vi "UDP Refresh Packet Sizes.vi"(8 "error in (no error)":errorcluster, 10 "UDP UI References in":T2, 11 "node References":T1) -> (0 "error out":errorcluster, 2 "UDP UI References out":T2, 3 "node References out":T1)   [LabVIEW 2015, in "E2E Tag Exchange editor node.lvclass"]
uses:
  E2E Tag Exchange editor node.lvclass
  UDP UI References.ctl
  object references.ctl
  <vilib>/NI/DCAF/Tag Editor Core/Configuration Editor/Classes/Engine Parent/Engine Parent Editor Node.lvclass
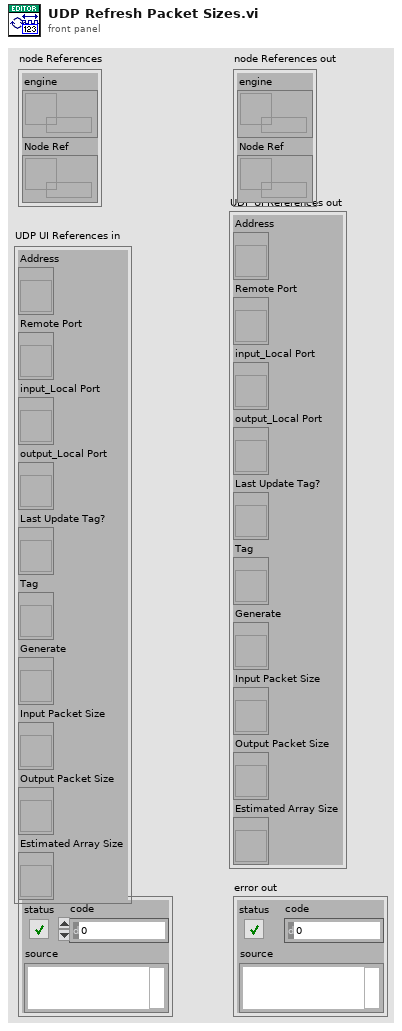
[diagram p1: front panel]
types:
  T1 = typedef "E2E Tag Exchange editor node.lvclass/object references.ctl" = cluster{"engine":refnum<data-value>, "Node Ref":refnum<data-value>}
  T2 = typedef "E2E Tag Exchange editor node.lvclass/UDP UI References.ctl" = cluster{"Address":refnum<vi>, "Remote Port":refnum<vi>, "input_Local Port":refnum<vi>, "output_Local Port":refnum<vi>, "Last Update Tag?":refnum<vi>, "Tag":refnum<vi>, "Generate":refnum<vi>, "Input Packet Size":refnum<vi>, "Output Packet Size":refnum<vi>, "Estimated Array Size":refnum<vi>}
  T3 = typedef "TBM channel.lvclass/data tables.ctl" = cluster{"input data":T4, "processing parameter":T4, "processing result":T4, "output data":T4}
  T4 = typedef "tag bus.lvlib/dictionary table pair.ctl" = cluster{"data dictionary":refnum<class "data dictionary.lvclass">, "data table":T5}
  T5 = typedef "tag bus.lvlib/data table.lvlib/data table.ctl" = cluster{"Double":dbl[], "Single":sgl[], "I64":i64[], "I32":i32[], "I16":i16[], "I8":i8[], "U64":u64[], "U32":u32[], "U16":u16[], "U8":u8[], "Boolean":bool[], "String":string[], "Array of Double":cluster{"DBL Array":dbl[]}[], "Array of Single":cluster{"SGL Array":sgl[]}[], "Array of I64":cluster{"I64 Array":i64[]}[], "Array of I32":cluster{"I32 Array":i32[]}[], "Array of I16":cluster{"I16 Array":i16[]}[], "Array of I8":cluster{"I8 Array":i8[]}[], "Array of U64":cluster{"U64 Array":u64[]}[], "Array of U32":cluster{"U32 Array":u32[]}[], "Array of U16":cluster{"U16 Array":u16[]}[], "Array of U8":cluster{"U8 Array":u8[]}[], "Array of Boolean":cluster{"Boolean Array":bool[]}[], "Array of String":cluster{"String Array":string[]}[]}
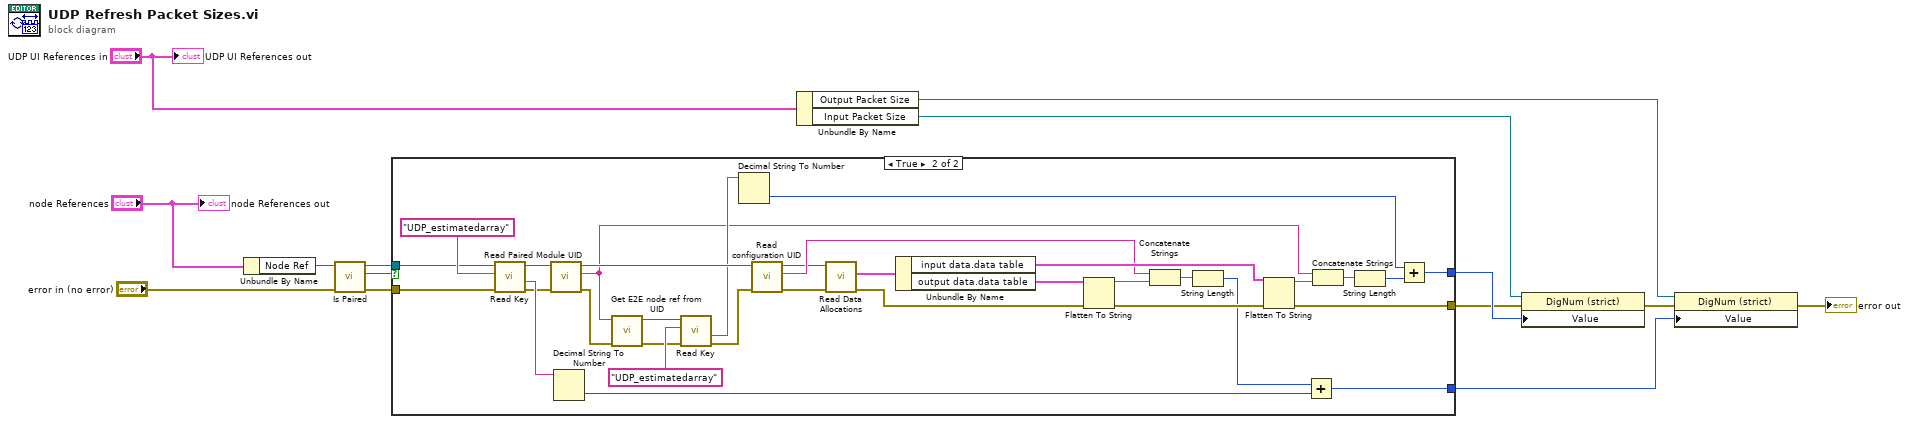
[diagram p0: block diagram]
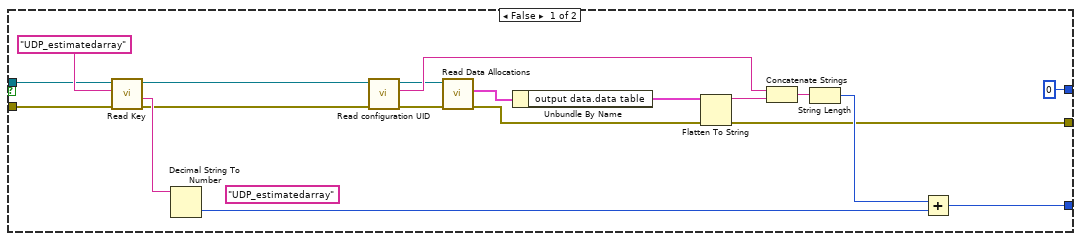
[diagram p2: hidden frame]
diagram:
  n1 = Unbundle By Name("node References") -> ("Node Ref"=w5:refnum<data-value>)
  n2 = call "Is Paired.vi"("error in (no error)"="error in (no error)", "E2E editor node in"=w5) -> ("error out"=w3:errorcluster, "Paired?"=w2:bool, "E2E editor node out"=w1:refnum<data-value>)  [unwired: 7 in]
  n3 = case shown="True" w2 {
    tunnel: [w26 w53] -> w12
    tunnel: [0 w50] -> w9
    tunnel: [w18 w65] -> w8
    tunnel: w3 -> [w22 w45]
    tunnel: w1 -> [w23 w46]
    frame False {
      (unwired) "UDP_estimatedarray" ("Key")
      n4 = call "Read Key.vi"("error in (no error)"=w22, "Key"="UDP_estimatedarray", "E2E editor node in"=w23) -> ("error out"=w15:errorcluster, "Value"=w25:string, "E2E editor node out"=w16:refnum<data-value>)  [unwired: 6 in]
      n5 = Decimal String To Number(string=w25) -> (number=w19:i32)  [unwired: 2 in, 1 out]
      n6 = call "Read configuration UID.vi"("error in (no error)"=w15, "E2E editor node in"=w16) -> ("error out"=w33:errorcluster, "Module UID"=w30:string, "E2E editor node out"=w29:refnum<data-value>)  [unwired: 7 in]
      n7 = call "Read Data Allocations.vi"("error in (no error)"=w33, "E2E editor node in"=w29) -> ("error out"=w21:errorcluster, "data allocations"=w32:T3)  [unwired: 7 in, 1 out]
      n8 = Unbundle By Name(w32) -> ("output data.data table"=w28:T5)
      n9 = Flatten To String(anything=w28, error in (no error)=w21) -> (data string=w27:string, error out=w18:errorcluster)  [unwired: 2 in, 1 out]
      n10 = Concatenate Strings(w30, w27) -> (w31:string)
      n11 = String Length(string=w31) -> (length=w20:i32)
      n12 = Add(x=w20, y=w19) -> (x+y=w26:i32)
    }
    frame True {
      n13 = call "Read Key.vi"("error in (no error)"=w45, "Key"="UDP_estimatedarray", "E2E editor node in"=w46) -> ("error out"=w49:errorcluster, "Value"=w52:string, "E2E editor node out"=w48:refnum<data-value>)  [unwired: 6 in]
      n14 = call "Read Paired Module UID.vi"("error in (no error)"=w49, "E2E editor node in"=w48) -> ("error out"=w44:errorcluster, "Paired Module UID"=w38:string, "E2E editor node out"=w47:refnum<data-value>)  [unwired: 7 in]
      n15 = Decimal String To Number(string=w52) -> (number=w34:i32)  [unwired: 2 in, 1 out]
      n16 = call "Get E2E node ref from UID.vi"("error in (no error)"=w44, "UID"=w38) -> ("error out"=w40:errorcluster, "E2E editor node ref"=w41:refnum<data-value>)  [unwired: 8 in]
      n17 = call "Read Key.vi"("error in (no error)"=w40, "Key"="UDP_estimatedarray", "E2E editor node in"=w41) -> ("error out"=w39:errorcluster, "Value"=w43:string)  [unwired: 6 in, 1 out]
      n18 = Decimal String To Number(string=w43) -> (number=w36:i32)  [unwired: 2 in, 1 out]
      n19 = call "Read configuration UID.vi"("error in (no error)"=w39, "E2E editor node in"=w47) -> ("error out"=w64:errorcluster, "Module UID"=w58:string, "E2E editor node out"=w57:refnum<data-value>)  [unwired: 7 in]
      n20 = call "Read Data Allocations.vi"("error in (no error)"=w64, "E2E editor node in"=w57) -> ("error out"=w37:errorcluster, "data allocations"=w63:T3)  [unwired: 7 in, 1 out]
      n21 = Unbundle By Name(w63) -> ("input data.data table"=w60:T5, "output data.data table"=w55:T5)
      n22 = Flatten To String(anything=w55, error in (no error)=w37) -> (data string=w54:string, error out=w59:errorcluster)  [unwired: 2 in, 1 out]
      n23 = Concatenate Strings(w58, w54) -> (w61:string)
      n24 = String Length(string=w61) -> (length=w35:i32)
      n25 = Flatten To String(anything=w60, error in (no error)=w59) -> (data string=w56:string, error out=w65:errorcluster)  [unwired: 2 in, 1 out]
      n26 = Add(x=w35, y=w34) -> (x+y=w53:i32)
      n27 = Concatenate Strings(w38, w56) -> (w62:string)
      n28 = String Length(string=w62) -> (length=w66:i32)
      n29 = Add(x=w36, y=w66) -> (x+y=w50:i32)
    }
  }
  n30 = Unbundle By Name("UDP UI References in") -> ("Output Packet Size"=w13:refnum<vi>, "Input Packet Size"=w10:refnum<vi>)
  n31 = property class="DigNum (strict)"(reference=w10, error in=w8, "Value"=w9) -> (error out=w11:errorcluster)  [unwired: 1 out]
  n32 = property class="DigNum (strict)"(reference=w13, error in=w11, "Value"=w12) -> (error out=→"error out":errorcluster)  [unwired: 1 out]
  "UDP UI References out" <- "UDP UI References in"
  "node References out" <- "node References"
